vi "Day 16.vi"() -> ()   [LabVIEW 2021]
panel:
  in  "Input Selection":string(combo)
  out "Return Value":u64
  out "Sum of Versions":u64
  out "Input":string
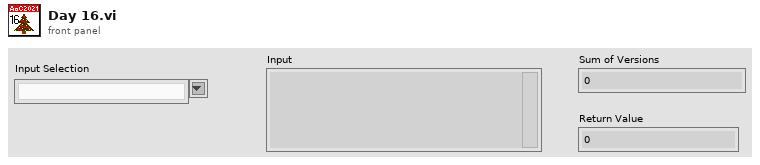
[diagram p1: front panel]
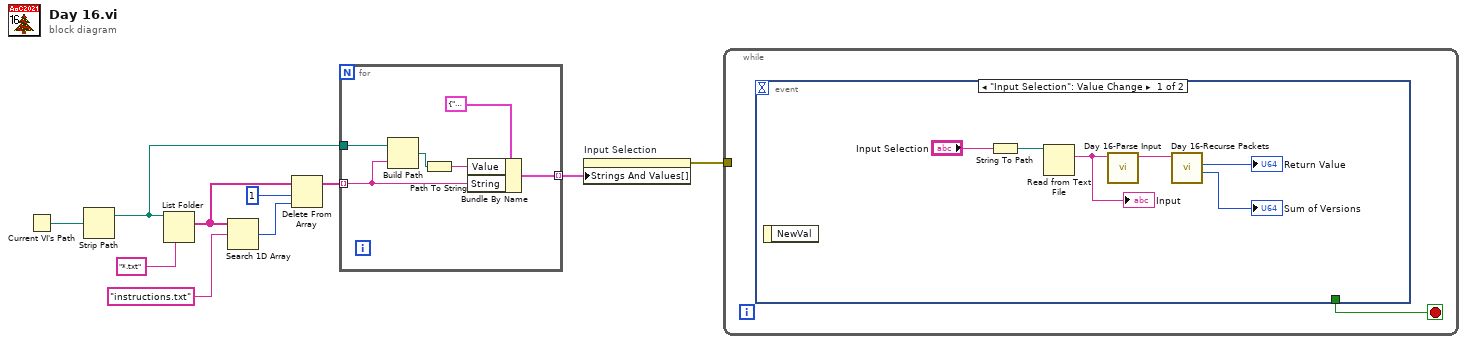
[diagram p0: block diagram]
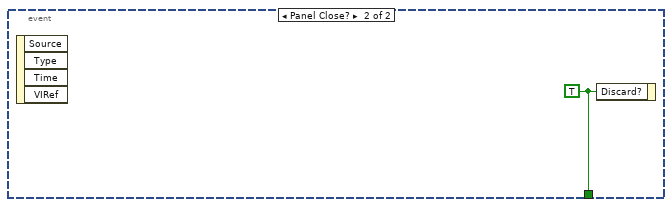
[diagram p2: hidden frame]
diagram:
  n1 = Current VI's Path() -> (path=w10:path)
  n2 = Strip Path(path=w10) -> (stripped path=w3:path)  [unwired: 1 out]
  n3 = List Folder(path=w3, pattern="*.txt") -> (filenames=w1:string[])  [unwired: 2 in, 3 out]
  n4 = Search 1D Array(1D array=w1, element="instructions.txt" ("pattern")) -> (index of element=w6:i32)  [unwired: 1 in]
  n5 = Delete From Array(array=w1, length=1, index=w6) -> (array with subset deleted=w4:string[])  [unwired: 1 out]
  n6 = for {
    tunnel: w4 -> [w14] mode=indexing
    tunnel: w3 -> [w15]
    tunnel: [w11] -> w2 mode=indexing
    n7 = Build Path(base path=w15, name or relative path=w14) -> (appended path=w13:path)
    n8 = Path To String(path=w13) -> (string=w12:string)
    n9 = Bundle By Name(cluster=cluster{"String":string, "Value":string} {"String"="", "Value"=""}, "Value"=w12, "String"=w14) -> (w11:cluster{"String":string, "Value":string})
  }
  n10 = property on="Input Selection" class="CmbBox"("Strings And Values[]"=w2) -> (error out=w8:errorcluster)  [unwired: 2 in, 1 out]
  n11 = while {
    tunnel: w8 -> [_]
    stop <- w17 stop-if-true
    n12 = event shown="[0] \"Input Selection\": Value Change" {
      selector: _ -> [_ _]
      dyn-events: _ -> [_ _]
      timeout: _ -> [_ _]
      tunnel: [_ w24] -> w17
      event "Input Selection": Value Change {
        n13 = event-data() -> ()  [unwired: 1 in, 1 out]
        n14 = String To Path(string="Input Selection") -> (path=w18:path)
        n15 = Read from Text File(file (use dialog)=w18) -> (text=w23:string)  [unwired: 3 in, 3 out]
        "Input" <- w23
        n16 = call "Day 16-Parse Input.vi"("String in"=w23) -> ("String out"=w22:string)  [unwired: 10 in]
        n17 = call "Day 16-Recurse Packets.vi"("String"=w22) -> ("Sum of Versions"=→"Sum of Versions":u64, "Return Value"=→"Return Value":u64)  [unwired: 8 in, 1 out]
      }
      event Panel Close? {
        w24 = TRUE ("Discard?")
        n18 = event-data() -> ()  [unwired: 1 in, 4 out]
        n19 = event-data("Discard?"=w24) -> ()  [unwired: 1 in, 1 out]
      }
    }
  }
